vi "LTE set RB Size.vi"(8 "error in (no error)":errorcluster caption="에러 입력(에러 없음)", 11 "Instrument Manager 입력":refnum<class "Instrument Manager.lvclass">) -> (0 "error out":errorcluster caption="에러 출력", 3 "Instrument Manager 출력":refnum<class "Instrument Manager.lvclass">)   [LabVIEW 2023, in "Instrument Manager.lvclass"]
uses:
  Instrument Manager.lvclass
  Instrument Manager.lvclass/Instrument Manager.ctl
  Module/ANRITSU Call Box/Type Definition/LTE RB Setting Params.ctl
  Module/ANRITSU Call Box/ANRITSU Call Box.lvlib
  Module/ANRITSU Call Box/Interface Class/Anritsu Call Box.lvclass
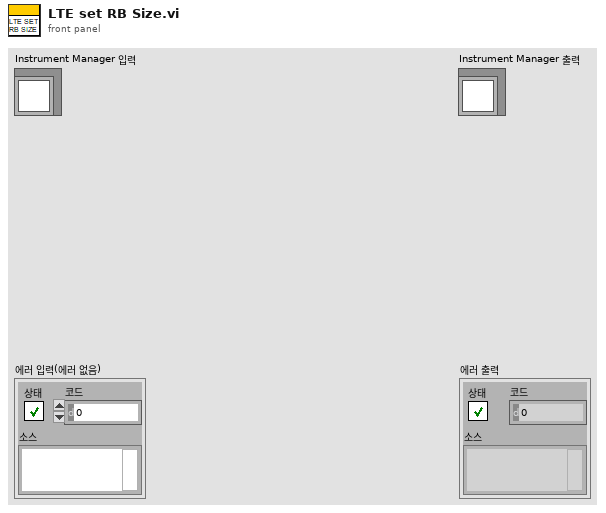
[diagram p1: front panel]
types:
  T1 = typedef "ANRITSU Call Box.lvlib/LTE RB Setting Params.ctl" = cluster{"RB Value":i32, "Target CA Type":enum16{"PCC", "SCC1"}, "RB Setting Type":enum16{"Number of RB", "Starting RB"}}
  T2 = cluster{"Anritsu Call Box":refnum<class "Anritsu Call Box.lvclass">, "Spectrum Analyzer":refnum<class "Interface_Spectrum.lvclass">, "RF Switch Box":refnum<class "RF Filter Box.lvclass">, "Turn Table":refnum<class "Interface - Turn Table.lvclass">, "Mast":refnum<class "Interface - Mast.lvclass">, "3D Controller":refnum<class "Interface_3D Controller.lvclass">}
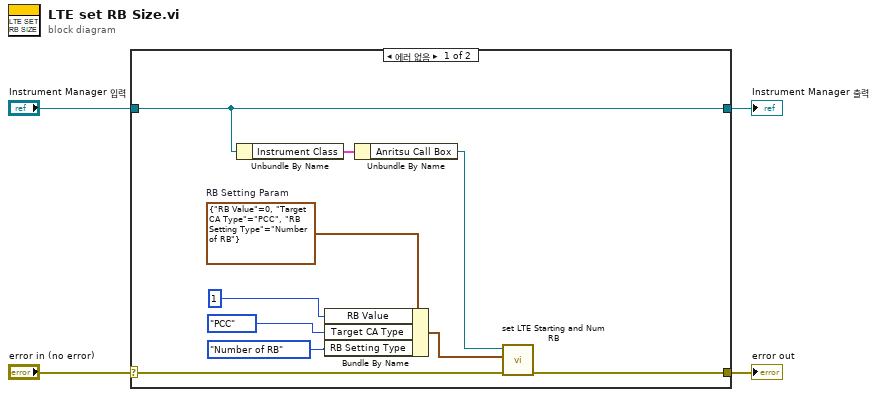
[diagram p0: block diagram]
diagram:
  n1 = case shown="에러 없음" "error in (no error)" {
    selector: "error in (no error)" -> [w9 w16]
    tunnel: [w8 w16] -> w3
    tunnel: [w7 w15] -> w1
    tunnel: "Instrument Manager 입력" -> [w7 w15]
    frame No Error {
      w14 = T1 {"RB Value"=0, "Target CA Type"=enum."PCC", "RB Setting Type"=enum."Number of RB"}  # RB Setting Param
      n2 = Unbundle By Name(w7) -> ("Instrument Class"=w6:T2)
      n3 = Bundle By Name(cluster=w14, "RB Value"=1, "Target CA Type"=enum16{"PCC", "SCC1"}."PCC", "RB Setting Type"=enum16{"Number of RB", "Starting RB"}."Number of RB") -> (w10:T1)
      n4 = Unbundle By Name(w6) -> ("Anritsu Call Box"=w5:refnum<class "Anritsu Call Box.lvclass">)
      n5 = call-dynamic "set LTE Starting and Num RB.vi"("error in (no error)"=w9, "RB Setting Param"=w10, "Anritsu Call Box in"=w5) -> ("error out"=w8:errorcluster)  [unwired: 7 in, 1 out]
    }
    frame Error {
    }
  }
  "error out" <- w3
  "Instrument Manager 출력" <- w1
